vi "Set VI Icon Text Layer.vi"(8 "error in (no error)":errorcluster, 10 "Text":T1={"Line 1 text"="", "Line 2 text"="a", "Line 3 text"="b", "Line 4 text"="c"}, 11 "VI in":refnum<vi>) -> (0 "error out":errorcluster, 3 "VI out":refnum<vi>)   [LabVIEW 2019, in "gRPC Template Creation Utility.lvlib"]
doc: "This example reads the current icon of a VI and updates it with an entirely new icon which primarily focuses on the Text Layer."
uses:
  gRPC Template Creation Utility.lvlib
  <vilib>/LabVIEW Icon API/API_Text.ctl
  <vilib>/LabVIEW Icon API/LabVIEW Icon API.lvlib
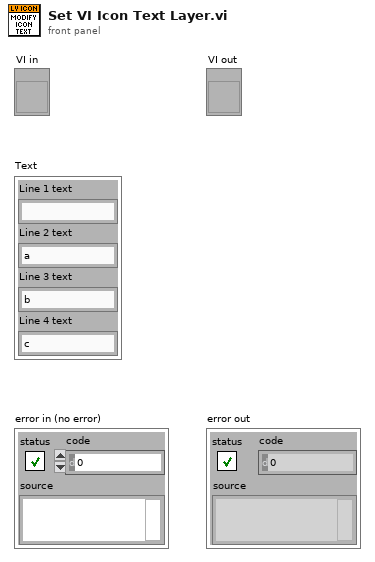
[diagram p1: front panel]
types:
  T1 = typedef "LabVIEW Icon API.lvlib/API_Text.ctl" = cluster{"Line 1 text":string, "Line 2 text":string, "Line 3 text":string, "Line 4 text":string}
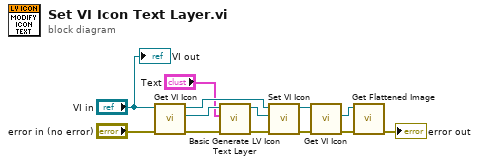
[diagram p0: block diagram]
diagram:
  n1 = call <vilib>:"Get VI Icon.vi"("error in (no error)"="error in (no error)", "VI Refnum in"="VI in") -> ("error out"=w3:errorcluster, "Icon"=w4:refnum<class "Icon.lvclass">, "VI Refnum out"=w13:refnum<vi>)  [unwired: 7 in]
  n2 = call "Basic Generate LV Icon Text Layer.vi"("error in (no error)"=w3, "Text"="Text", "Icon"=w4) -> ("error out"=w12:errorcluster, "Icon.lvlclass out"=w11:refnum<class "Icon.lvclass">)  [unwired: 7 in]
  n3 = call <vilib>:"Set VI Icon.vi"("error in (no error)"=w12, "Icon"=w11, "VI Refnum in"=w13) -> ("error out"=w10:errorcluster, "VI Refnum out"=w9:refnum<vi>)  [unwired: 7 in]
  n4 = call <vilib>:"Get VI Icon.vi"("error in (no error)"=w10, "VI Refnum in"=w9) -> ("error out"=w8:errorcluster, "Icon"=w7:refnum<class "Icon.lvclass">)  [unwired: 7 in, 1 out]
  n5 = call <vilib>:"Get Flattened Image.vi"("error in (no error)"=w8, "lv_icon.lvlib:Icon.lvclass in"=w7) -> ("error out"=→"error out":errorcluster)  [unwired: 6 in, 3 out]
  "VI out" <- "VI in"
